vi "Scale_Graph_X (SubVI).vi"(9 "Array":dbl[](array[numeric]), 10 "Übersetzung ermitteln aus":u8, 11 "XYGraph (Eingang)":refnum<vi>) -> (0 "xMax (Ausgang)":dbl, 1 "xMin (Ausgang)":dbl)   [LabVIEW 2014]
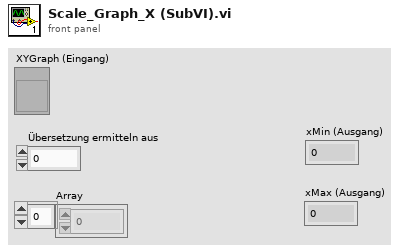
[diagram p1: front panel]
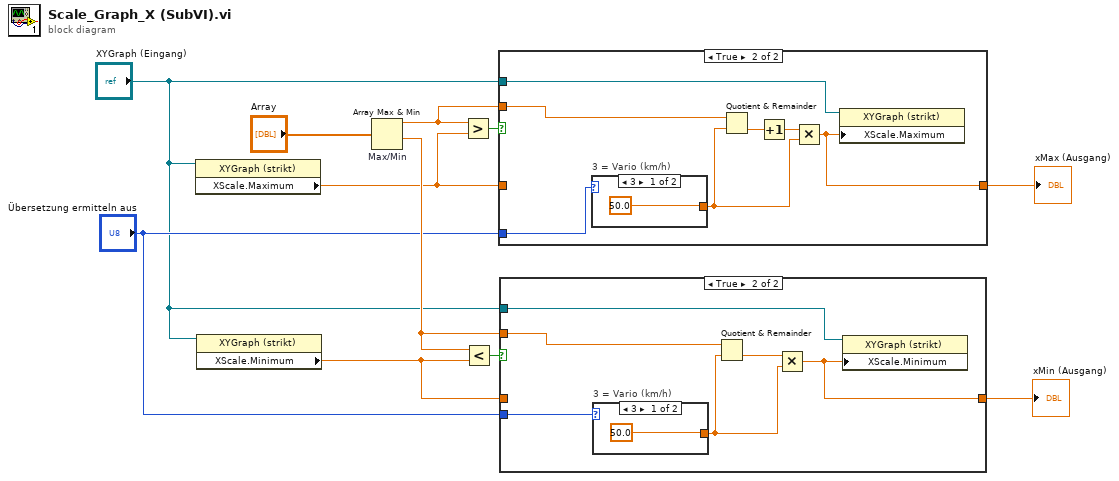
[diagram p0: block diagram]
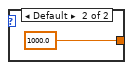
[diagram p3: hidden frame]
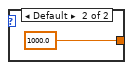
[diagram p5: hidden frame]
diagram:
  n1 = property on="Eigenschaftsknoten" class="XYGraph (strikt)"(reference="XYGraph (Eingang)") -> ("XScale.Maximum"=w2:dbl)  [unwired: 1 in, 2 out]
  n2 = property on="Eigenschaftsknoten" class="XYGraph (strikt)"(reference="XYGraph (Eingang)") -> ("XScale.Minimum"=w1:dbl)  [unwired: 1 in, 2 out]
  n3 = Array Max & Min "Max/Min"(array="Array") -> (max value=w9:dbl, min value=w7:dbl)  [unwired: 2 out]
  n4 = Greater?(x=w9, y=w2) -> (0:w10:bool)
  n5 = Less?(x=w7, y=w1) -> (x < y?=w8:bool)
  n6 = case shown="True" w10 {
    tunnel: w9 -> [_ w16]
    tunnel: "XYGraph (Eingang)" -> [_ w17]
    tunnel: "Übersetzung ermitteln aus" -> [_ w14]
    tunnel: [w12 w13] -> w4
    tunnel: w2 -> [w12 _]
    frame False {
    }
    frame True {
      n7 = case "3 = Vario (km/h)" shown="3" w14 {
        tunnel: [50.0 1000.0] -> w15
        frame 3 {
        }
        frame Default {
        }
      }
      n8 = Quotient & Remainder(x=w16, y=w15) -> (floor(x/y)=w18:dbl)  [unwired: 1 out]
      n9 = Increment(x=w18) -> (x+1=w19:dbl)
      n10 = Multiply(x=w19, y=w15) -> (x*y=w13:dbl)
      n11 = property on="Eigenschaftsknoten" class="XYGraph (strikt)"(reference=w17, "XScale.Maximum"=w13) -> ()  [unwired: 1 in, 2 out]
    }
  }
  "xMax (Ausgang)" <- w4
  n12 = case shown="True" w8 {
    tunnel: w7 -> [_ w27]
    tunnel: "XYGraph (Eingang)" -> [_ w28]
    tunnel: "Übersetzung ermitteln aus" -> [_ w25]
    tunnel: [w22 w23] -> w3
    tunnel: w1 -> [w22 _]
    frame False {
    }
    frame True {
      n13 = case "3 = Vario (km/h)" shown="3" w25 {
        tunnel: [50.0 1000.0] -> w26
        frame 3 {
        }
        frame Default {
        }
      }
      n14 = Quotient & Remainder(x=w27, y=w26) -> (floor(x/y)=w24:dbl)  [unwired: 1 out]
      n15 = Multiply(x=w24, y=w26) -> (x*y=w23:dbl)
      n16 = property on="Eigenschaftsknoten" class="XYGraph (strikt)"(reference=w28, "XScale.Minimum"=w23) -> ()  [unwired: 1 in, 2 out]
    }
  }
  "xMin (Ausgang)" <- w3
